vi "Validate Configurable Sequence.vi"(8 "error in":errorcluster, 10 "IO List":cluster{"name":string, "type":string}[](array[cluster]), 11 "Configurable Sequence":T1) -> (0 "error out":errorcluster, 3 "problem":string)   [LabVIEW 2026]
doc: "Checks every IO name used by a configurable sequence against the rig IO list and its type. Returns error 5002 naming the first problem. AF-free."
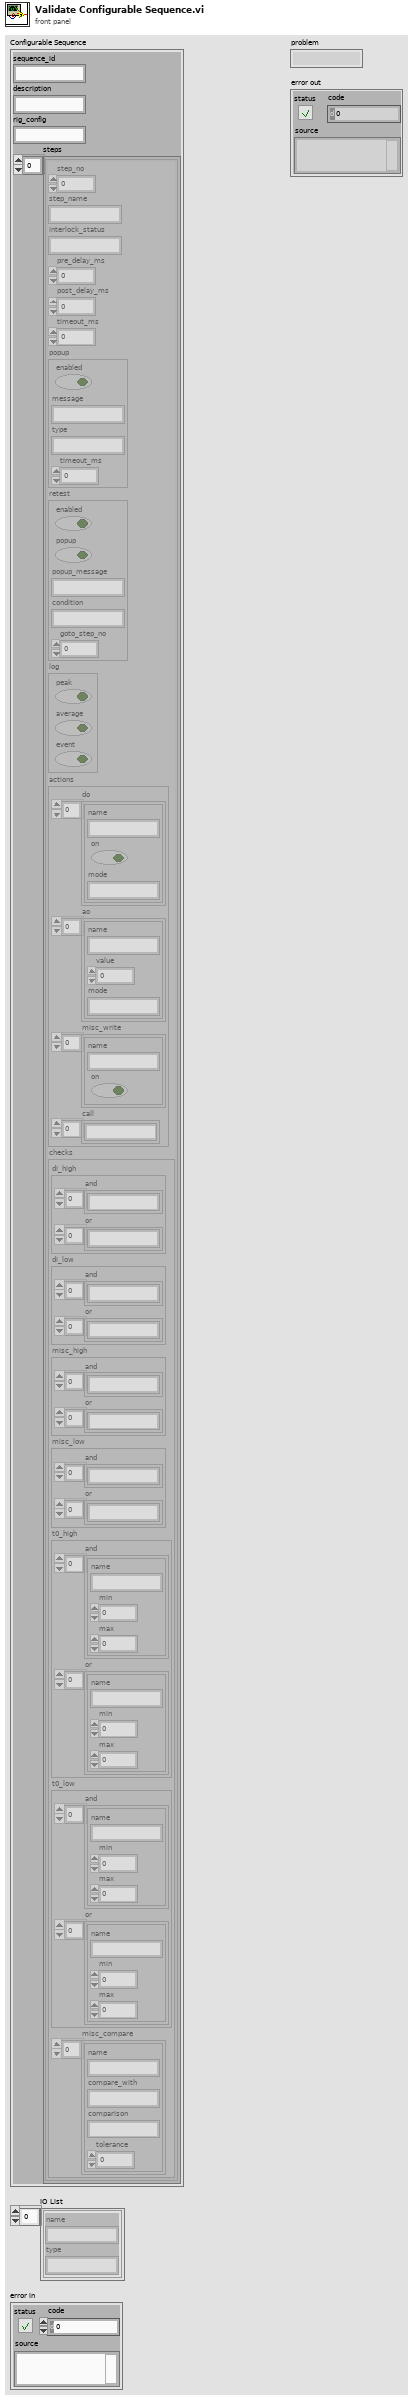
[diagram p1: front panel]
types:
  T1 = cluster{"sequence_id":string, "description":string, "rig_config":string, "steps":cluster{"step_no":i32, "step_name":string, "interlock_status":string, "pre_delay_ms":dbl, "post_delay_ms":dbl, "timeout_ms":dbl, "popup":cluster{"enabled":bool, "message":string, "type":string, "timeout_ms":dbl}, "retest":cluster{"enabled":bool, "popup":bool, "popup_message":string, "condition":string, "goto_step_no":i32}, "log":cluster{"peak":bool, "average":bool, "event":bool}, "actions":cluster{"do":cluster{"name":string, "on":bool, "mode":string}[], "ao":cluster{"name":string, "value":dbl, "mode":string}[], "misc_write":cluster{"name":string, "on":bool}[], "call":string[]}, "checks":cluster{"di_high":cluster{"and":string[], "or":string[]}, "di_low":cluster{"and":string[], "or":string[]}, "misc_high":cluster{"and":string[], "or":string[]}, "misc_low":cluster{"and":string[], "or":string[]}, "t0_high":cluster{"and":cluster{"name":string, "min":dbl, "max":dbl}[], "or":cluster{"name":string, "min":dbl, "max":dbl}[]}, "t0_low":cluster{"and":cluster{"name":string, "min":dbl, "max":dbl}[], "or":cluster{"name":string, "min":dbl, "max":dbl}[]}, "misc_compare":cluster{"name":string, "compare_with":string, "comparison":string, "tolerance":dbl}[]}}[]}
  T2 = cluster{"step_no":i32, "step_name":string, "interlock_status":string, "pre_delay_ms":dbl, "post_delay_ms":dbl, "timeout_ms":dbl, "popup":cluster{"enabled":bool, "message":string, "type":string, "timeout_ms":dbl}, "retest":cluster{"enabled":bool, "popup":bool, "popup_message":string, "condition":string, "goto_step_no":i32}, "log":cluster{"peak":bool, "average":bool, "event":bool}, "actions":cluster{"do":cluster{"name":string, "on":bool, "mode":string}[], "ao":cluster{"name":string, "value":dbl, "mode":string}[], "misc_write":cluster{"name":string, "on":bool}[], "call":string[]}, "checks":cluster{"di_high":cluster{"and":string[], "or":string[]}, "di_low":cluster{"and":string[], "or":string[]}, "misc_high":cluster{"and":string[], "or":string[]}, "misc_low":cluster{"and":string[], "or":string[]}, "t0_high":cluster{"and":cluster{"name":string, "min":dbl, "max":dbl}[], "or":cluster{"name":string, "min":dbl, "max":dbl}[]}, "t0_low":cluster{"and":cluster{"name":string, "min":dbl, "max":dbl}[], "or":cluster{"name":string, "min":dbl, "max":dbl}[]}, "misc_compare":cluster{"name":string, "compare_with":string, "comparison":string, "tolerance":dbl}[]}}[]
  T3 = cluster{"do":cluster{"name":string, "on":bool, "mode":string}[], "ao":cluster{"name":string, "value":dbl, "mode":string}[], "misc_write":cluster{"name":string, "on":bool}[], "call":string[]}
  T4 = cluster{"di_high":cluster{"and":string[], "or":string[]}, "di_low":cluster{"and":string[], "or":string[]}, "misc_high":cluster{"and":string[], "or":string[]}, "misc_low":cluster{"and":string[], "or":string[]}, "t0_high":cluster{"and":cluster{"name":string, "min":dbl, "max":dbl}[], "or":cluster{"name":string, "min":dbl, "max":dbl}[]}, "t0_low":cluster{"and":cluster{"name":string, "min":dbl, "max":dbl}[], "or":cluster{"name":string, "min":dbl, "max":dbl}[]}, "misc_compare":cluster{"name":string, "compare_with":string, "comparison":string, "tolerance":dbl}[]}
  T5 = cluster{"and":cluster{"name":string, "min":dbl, "max":dbl}[], "or":cluster{"name":string, "min":dbl, "max":dbl}[]}
  T6 = cluster{"name":string, "compare_with":string, "comparison":string, "tolerance":dbl}[]
  T7 = cluster{"name":string, "on":bool, "mode":string}[]
  T8 = cluster{"name":string, "value":dbl, "mode":string}[]
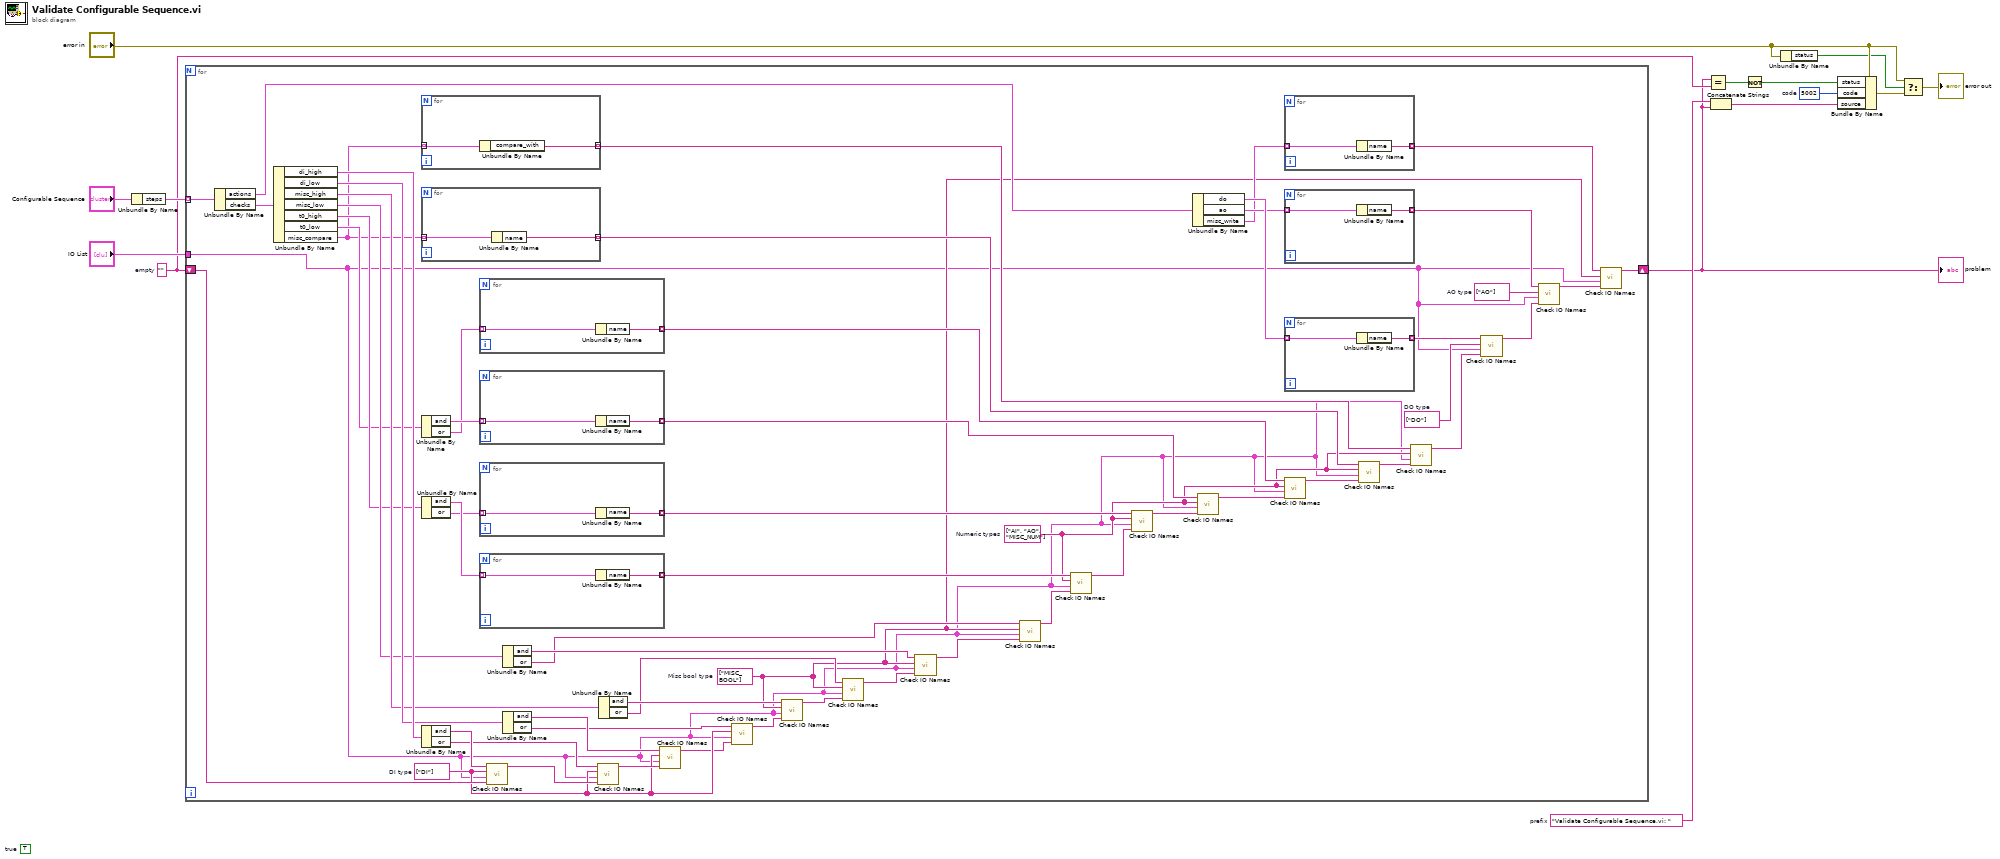
[diagram p0: block diagram]
diagram:
  (unwired) TRUE  # true
  w10 = "Validate Configurable Sequence.vi: "  # prefix
  w7 = 5002  # code
  w11 = ""  # empty
  n1 = Unbundle By Name("Configurable Sequence") -> ("steps"=w13:T2)
  n2 = for {
    tunnel: w13 -> [w72] mode=indexing
    tunnel: "IO List" -> [w17]
    shift-right: [w15] -> w2
    shift-left: w11 -> [w67]
    w30 = string[] ["AI", "AO", "MISC_NUM"]  # Numeric types
    w18 = string[] ["MISC_BOOL"]  # Misc bool type
    w22 = string[] ["AO"]  # AO type
    w26 = string[] ["DO"]  # DO type
    w60 = string[] ["DI"]  # DI type
    n3 = Unbundle By Name(w72) -> ("actions"=w71:T3, "checks"=w70:T4)
    n4 = Unbundle By Name(w70) -> ("di_high"=w69:cluster{"and":string[], "or":string[]}, "di_low"=w64:cluster{"and":string[], "or":string[]}, "misc_high"=w58:cluster{"and":string[], "or":string[]}, "misc_low"=w53:cluster{"and":string[], "or":string[]}, "t0_high"=w48:T5, "t0_low"=w41:T5, "misc_compare"=w32:T6)
    n5 = for {
      tunnel: w32 -> [w80] mode=indexing
      tunnel: [w79] -> w31 mode=indexing
      n6 = Unbundle By Name(w80) -> ("compare_with"=w79:string)
    }
    n7 = for {
      tunnel: w32 -> [w82] mode=indexing
      tunnel: [w81] -> w34 mode=indexing
      n8 = Unbundle By Name(w82) -> ("name"=w81:string)
    }
    n9 = Unbundle By Name(w41) -> ("and"=w40:cluster{"name":string, "min":dbl, "max":dbl}[], "or"=w37:cluster{"name":string, "min":dbl, "max":dbl}[])
    n10 = Unbundle By Name(w48) -> ("and"=w47:cluster{"name":string, "min":dbl, "max":dbl}[], "or"=w44:cluster{"name":string, "min":dbl, "max":dbl}[])
    n11 = Unbundle By Name(w69) -> ("and"=w68:string[], "or"=w66:string[])
    n12 = for {
      tunnel: w37 -> [w84] mode=indexing
      tunnel: [w83] -> w36 mode=indexing
      n13 = Unbundle By Name(w84) -> ("name"=w83:string)
    }
    n14 = for {
      tunnel: w40 -> [w86] mode=indexing
      tunnel: [w85] -> w39 mode=indexing
      n15 = Unbundle By Name(w86) -> ("name"=w85:string)
    }
    n16 = for {
      tunnel: w44 -> [w88] mode=indexing
      tunnel: [w87] -> w43 mode=indexing
      n17 = Unbundle By Name(w88) -> ("name"=w87:string)
    }
    n18 = for {
      tunnel: w47 -> [w90] mode=indexing
      tunnel: [w89] -> w46 mode=indexing
      n19 = Unbundle By Name(w90) -> ("name"=w89:string)
    }
    n20 = call "Check IO Names.vi"("prior problem"=w67, "IO List"=w17, "allowed types"=w60, "names"=w68) -> ("problem"=w65:string)  [unwired: 7 in]
    n21 = Unbundle By Name(w53) -> ("and"=w52:string[], "or"=w50:string[])
    n22 = Unbundle By Name(w64) -> ("and"=w63:string[], "or"=w61:string[])
    n23 = call "Check IO Names.vi"("prior problem"=w65, "IO List"=w17, "allowed types"=w60, "names"=w66) -> ("problem"=w62:string)  [unwired: 7 in]
    n24 = Unbundle By Name(w58) -> ("and"=w57:string[], "or"=w55:string[])
    n25 = call "Check IO Names.vi"("prior problem"=w62, "IO List"=w17, "allowed types"=w60, "names"=w63) -> ("problem"=w59:string)  [unwired: 7 in]
    n26 = call "Check IO Names.vi"("prior problem"=w59, "IO List"=w17, "allowed types"=w60, "names"=w61) -> ("problem"=w56:string)  [unwired: 7 in]
    n27 = call "Check IO Names.vi"("prior problem"=w56, "IO List"=w17, "allowed types"=w18, "names"=w57) -> ("problem"=w54:string)  [unwired: 7 in]
    n28 = call "Check IO Names.vi"("prior problem"=w54, "IO List"=w17, "allowed types"=w18, "names"=w55) -> ("problem"=w51:string)  [unwired: 7 in]
    n29 = call "Check IO Names.vi"("prior problem"=w51, "IO List"=w17, "allowed types"=w18, "names"=w52) -> ("problem"=w49:string)  [unwired: 7 in]
    n30 = call "Check IO Names.vi"("prior problem"=w49, "IO List"=w17, "allowed types"=w18, "names"=w50) -> ("problem"=w45:string)  [unwired: 7 in]
    n31 = call "Check IO Names.vi"("prior problem"=w45, "IO List"=w17, "allowed types"=w30, "names"=w46) -> ("problem"=w42:string)  [unwired: 7 in]
    n32 = call "Check IO Names.vi"("prior problem"=w42, "IO List"=w17, "allowed types"=w30, "names"=w43) -> ("problem"=w38:string)  [unwired: 7 in]
    n33 = Unbundle By Name(w71) -> ("do"=w28:T7, "ao"=w24:T8, "misc_write"=w20:cluster{"name":string, "on":bool}[])
    n34 = call "Check IO Names.vi"("prior problem"=w38, "IO List"=w17, "allowed types"=w30, "names"=w39) -> ("problem"=w35:string)  [unwired: 7 in]
    n35 = for {
      tunnel: w20 -> [w74] mode=indexing
      tunnel: [w73] -> w19 mode=indexing
      n36 = Unbundle By Name(w74) -> ("name"=w73:string)
    }
    n37 = for {
      tunnel: w24 -> [w76] mode=indexing
      tunnel: [w75] -> w23 mode=indexing
      n38 = Unbundle By Name(w76) -> ("name"=w75:string)
    }
    n39 = for {
      tunnel: w28 -> [w78] mode=indexing
      tunnel: [w77] -> w27 mode=indexing
      n40 = Unbundle By Name(w78) -> ("name"=w77:string)
    }
    n41 = call "Check IO Names.vi"("prior problem"=w35, "IO List"=w17, "allowed types"=w30, "names"=w36) -> ("problem"=w33:string)  [unwired: 7 in]
    n42 = call "Check IO Names.vi"("prior problem"=w33, "IO List"=w17, "allowed types"=w30, "names"=w34) -> ("problem"=w29:string)  [unwired: 7 in]
    n43 = call "Check IO Names.vi"("prior problem"=w29, "IO List"=w17, "allowed types"=w30, "names"=w31) -> ("problem"=w25:string)  [unwired: 7 in]
    n44 = call "Check IO Names.vi"("prior problem"=w25, "IO List"=w17, "allowed types"=w26, "names"=w27) -> ("problem"=w21:string)  [unwired: 7 in]
    n45 = call "Check IO Names.vi"("prior problem"=w21, "IO List"=w17, "allowed types"=w22, "names"=w23) -> ("problem"=w16:string)  [unwired: 7 in]
    n46 = call "Check IO Names.vi"("prior problem"=w16, "IO List"=w17, "allowed types"=w18, "names"=w19) -> ("problem"=w15:string)  [unwired: 7 in]
  }
  "problem" <- w2
  n47 = Equal?(x=w2, y=w11) -> (x = y?=w9:bool)
  n48 = Concatenate Strings(w10, w2) -> (w6:string)
  n49 = Not(x=w9) -> (.not. x?=w8:bool)
  n50 = Unbundle By Name("error in") -> ("status"=w4:bool)
  n51 = Bundle By Name(cluster="error in", "status"=w8, "code"=w7, "source"=w6) -> (w3:errorcluster)
  n52 = Select(t="error in", s=w4, f=w3) -> (s? t:f=→"error out":errorcluster)
